vi "PostInstall.vi"(0 "Variant":variant) -> (15 "error out":errorcluster)   [LabVIEW 2026]
doc: "lvpm test fixture: package post-install hook. Reads the Package Name attribute of the Variant control as a string (empty string when the attribute is missing) and writes it to lvpm-test-hook-marker.txt in the system temporary directory, replacing any previous content. Shows no dialog and returns immediately; any file error is reported in error out."
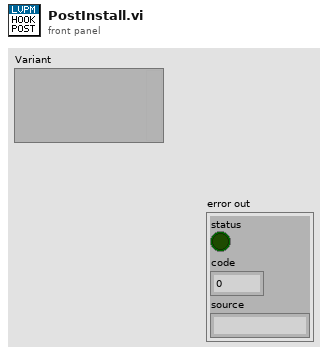
[diagram p1: front panel]
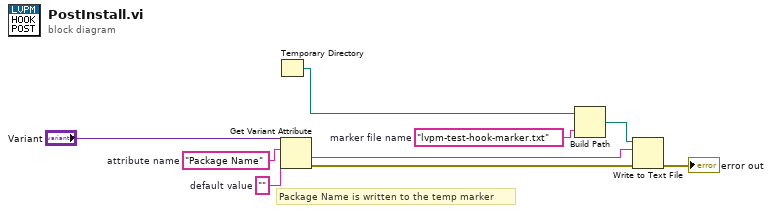
[diagram p0: block diagram]
diagram:
  w7 = "lvpm-test-hook-marker.txt"  # marker file name
  w3 = ""  # default value
  w2 = "Package Name"  # attribute name
  # "Package Name is written to the temp marker"
  n1 = Temporary Directory() -> (w6:path)
  n2 = Get Variant Attribute(Variant="Variant", name=w2, default value (empty Variant)=w3) -> (value=w4:string, error out=w5:errorcluster)  [unwired: 1 in, 2 out]
  n3 = Build Path(base path=w6, name or relative path=w7) -> (appended path=w8:path)
  n4 = Write to Text File(file (use dialog)=w8, text=w4, error in=w5) -> (error out=→"error out":errorcluster)  [unwired: 1 in, 2 out]
